vi "Lab06_task4_Aliasing.vi"() -> ()   [LabVIEW 2022 SP3]
uses:
  <vilib>/DAQmx/read.llb/DAQmx Read (Analog 2D DBL NChan NSamp).vi
  <vilib>/DAQmx/create/channels.llb/DAQmx Create Channel (AI-Voltage-Basic).vi
  <vilib>/DAQmx/configure/timing.llb/DAQmx Timing (Sample Clock).vi
  <vilib>/DAQmx/miscellaneous.llb/DAQmx Fill In Error Info.vi
  <vilib>/Utility/file.llb/Write Delimited Spreadsheet (DBL).vi
  <vilib>/express/express analysis/Spectral/Block/exnSpectralBlock spectral measurements RMS poly.vi
  <vilib>/express/express analysis/Spectral/Block/exnSpectralBlock spectral measurements RMS DDT.vi
  <vilib>/express/express analysis/Spectral/XNode/ExpressSpectralMeasurementsBlockNode.xnode
panel:
  out "Waveform Graph 2":dynamicdata(graph)
  in  "file path (dialog if empty)":path
  out "data":dbl[][](array[numeric]) format="%0.2f"
  out "error out":errorcluster
  out "Waveform Graph":dbl[][](graph)
  in  "number of samples per channel":i32=-1
  in  "samples per channel":i32=1000
  in  "rate":dbl=1000.0 format="%0.2f"
  in  "physical channels":tag
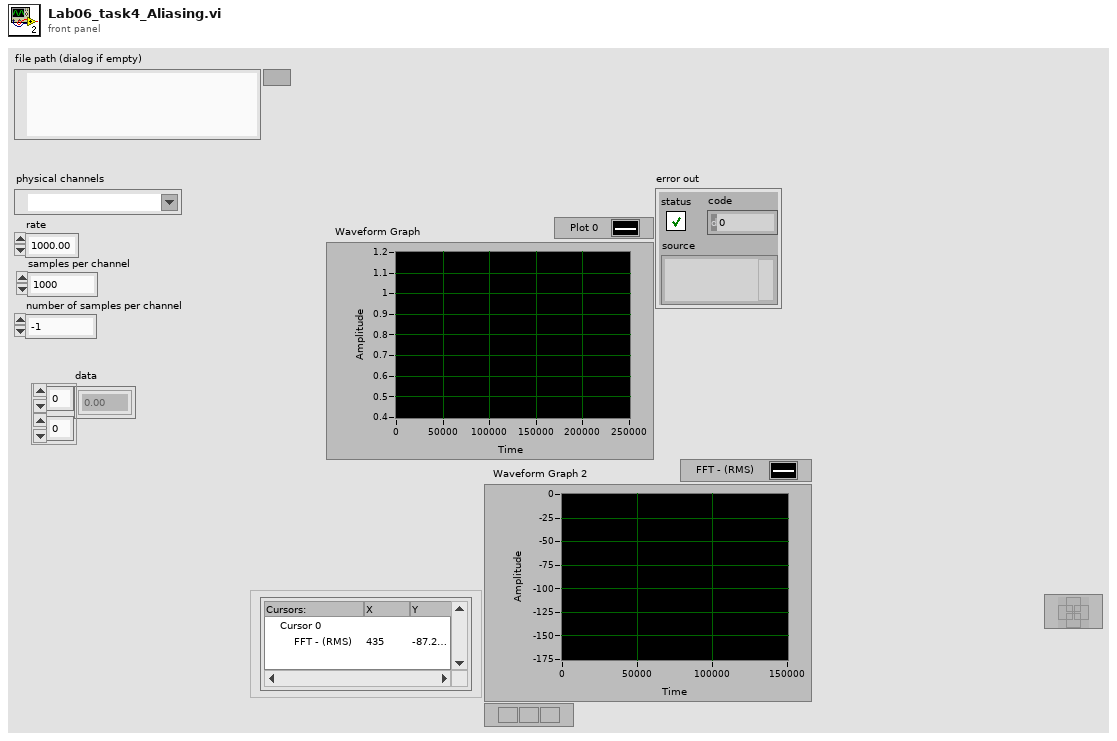
[diagram p1: front panel]
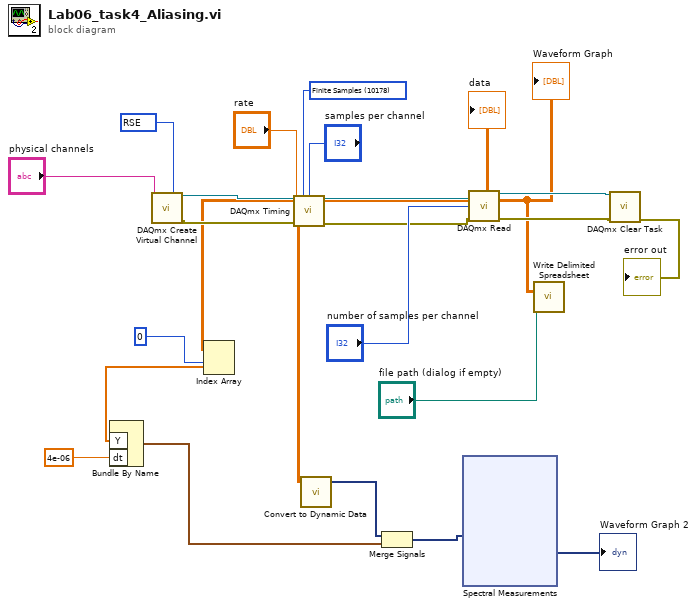
[diagram p0: block diagram]
diagram:
  w10 = 10083 items=["Default"=-1, "RSE"=10083, "NRSE"=10078, "Differential"=10106, "Pseudodifferential"=12529] ("input terminal configuration")
  w19 = 10178 items=["Finite Samples"=10178, "Continuous Samples"=10123, "Hardware Timed Single Point"=12522] ("sample mode")
  n1 = call-poly <vilib>:"DAQmx Create Virtual Channel.vi"("input terminal configuration"=w10, "physical channels"="physical channels") -> ("task out"=w21:refnum<k21>, "error out"=w14:errorcluster)  [unwired: 12 in]
  n2 = call-poly <vilib>:"DAQmx Timing.vi"("task/channels in"=w21, "sample mode"=w19, "samples per channel"="samples per channel", "rate"="rate", "error in"=w14) -> ("task out"=w17:refnum<k21>, "error out"=w13:errorcluster)  [unwired: 9 in]
  n3 = call-poly <vilib>:"DAQmx Read.vi"("task/channels in"=w17, "number of samples per channel"="number of samples per channel", "error in"=w13) -> ("task out"=w15:refnum<k21>, "data"=w6:dbl[][], "error out"=w12:errorcluster)  [unwired: 10 in]
  "Waveform Graph" <- w6
  "data" <- w6
  n4 = Index Array(array=w6, index (row)=0) -> (element=w4:dbl[])  [unwired: 1 in]
  n5 = Bundle By Name("Y"=w4, "dt"=4e-06) -> (w1:waveform(dbl))  [unwired: 1 in]
  n6 = call "Convert to Dynamic Data"("2D Array"=w6) -> ("Dynamic Data Type"=w8:dynamicdata)  [unwired: 3 in]
  n7 = Merge Signals(w8, w1) -> (w2:dynamicdata)
  n8 = xnode "Spectral Measurements"("Signals"=w2) -> ("FFT - (RMS)"=→"Waveform Graph 2":dynamicdata)  [unwired: 1 in, 2 out]
  n9 = call-poly <vilib>:"Write Delimited Spreadsheet.vi"("file path (dialog if empty)"="file path (dialog if empty)", "2D data"=w6) -> ()  [unwired: 12 in, 2 out]
  n10 = call <vilib>:"DAQmx Clear Task.vi"("task in"=w15, "error in"=w12) -> ("error out"=→"error out":errorcluster)  [unwired: 13 in]
